vi "[ex ce] Simple Waveform Processing.vi"() -> ()   [LabVIEW 2021]
doc: "In this example, CalcExpress.vi is used for simple processing of waveform signals.\n\n::: CalcExpress Toolkit :::\nCopyright (c) 2000-2026 Konstantin Shifershteyn. All rights reserved."
uses:
  <vilib>/measure/NI_MABase.lvlib
panel:
  out "Output signals":waveform(dbl)[](graph)
  in  "Expression":string="Out1 = (In1 + In2) / 2;  // calculate average of two input signals\nOut2 = (Out1 > 1.25);    // compare the average with a threshold\n\nOut3 = (In1 > In2);      // compare two signals\nOut3 -= 2;               // substract 2 from Out3"
  out "Input signals":waveform(dbl)[](graph)
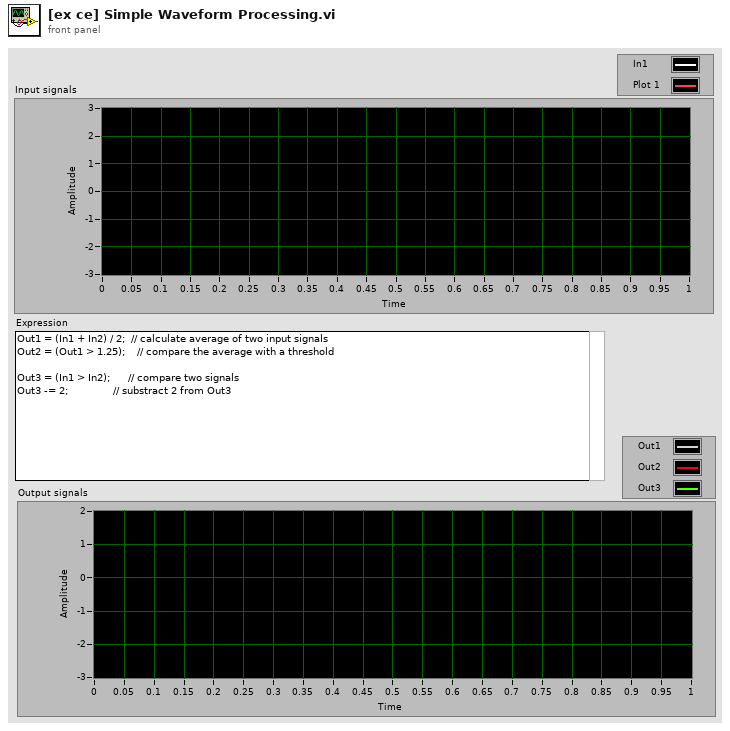
[diagram p1: front panel]
types:
  T1 = typedef "VarMan Variable Context Handle.ctl" = i32
  T2 = enum16{"create", "destroy", "set value", "get value"}
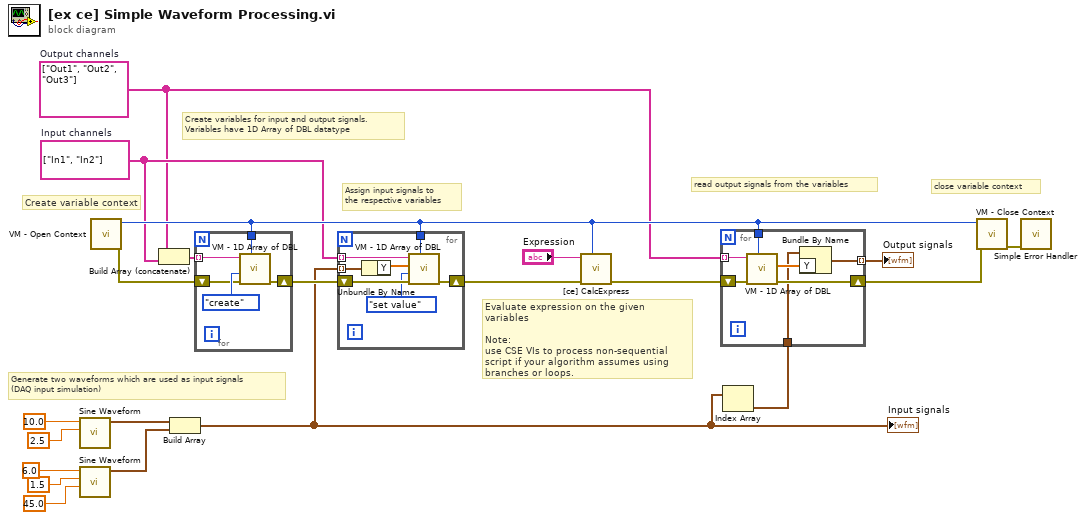
[diagram p0: block diagram]
diagram:
  w7 = string[] ["Out1", "Out2", "Out3"]  # Output channels
  w9 = string[] ["In1", "In2"]  # Input channels
  # "Create variables for input and output signals.\nVariables have 1D Array of DBL datatype"
  # "Evaluate expression on the given variables\n\nNote:\nuse CSE VIs to process non-sequential\nscript if your algorithm assumes using\nbranches or loops."
  # "close variable context"
  # "read output signals from the variables"
  # "Assign input signals to\nthe respective variables"
  # "Create variable context"
  # "Generate two waveforms which are used as input signals\n(DAQ input simulation)"
  n1 = call <vilib>:"Sine Waveform.vi"("amplitude"=2.5, "frequency"=10.0) -> ("signal out"=w16:waveform(dbl))  [unwired: 8 in, 1 out]
  n2 = call <vilib>:"Sine Waveform.vi"("phase"=45.0, "amplitude"=1.5, "frequency"=6.0) -> ("signal out"=w13:waveform(dbl))  [unwired: 7 in, 1 out]
  n3 = call "VM - Open Context.vi"() -> ("error out"=w20:errorcluster, "VC Handle out"=w11:T1)  [unwired: 9 in, 1 out]
  n4 = Build Array (concatenate)(w7, w9) -> (w8:string[])
  n5 = Build Array(w16, w13) -> (w4:waveform(dbl)[])
  "Input signals" <- w4
  n6 = for {
    shift-right: [w24] -> w14
    shift-left: w20 -> [w25]
    tunnel: w11 -> [w23]
    tunnel: w8 -> [w22] mode=indexing
    n7 = call "VM - 1D Array of DBL.vi"("VC Handle"=w23, "error in"=w25, "cmd"=T2."create", "name_spec"=w22) -> ("error out"=w24:errorcluster)  [unwired: 2 in, 5 out]
  }
  n8 = for {
    tunnel: w11 -> [w31]
    shift-right: [w30] -> w10
    shift-left: w14 -> [w33]
    tunnel: w9 -> [w29] mode=indexing
    tunnel: w4 -> [w27] mode=indexing
    n9 = Unbundle By Name(w27) -> ("Y"=w28:dbl[])
    n10 = call "VM - 1D Array of DBL.vi"("VC Handle"=w31, "error in"=w33, "cmd"=T2."set value", "value in"=w28, "name_spec"=w29) -> ("error out"=w30:errorcluster)  [unwired: 1 in, 5 out]
  }
  n11 = call "[ce] CalcExpress.vi"("VC Handle"=w11, "error in"=w10, "expression"="Expression") -> ("error out"=w12:errorcluster)  [unwired: 3 in, 3 out]
  n12 = Index Array(array=w4) -> (element=w3:waveform(dbl))  [unwired: 1 in]
  n13 = for {
    tunnel: w11 -> [w39]
    shift-right: [w37] -> w6
    shift-left: w12 -> [w40]
    tunnel: w7 -> [w36] mode=indexing
    tunnel: [w35] -> w5 mode=indexing
    tunnel: w3 -> [w34]
    n14 = call "VM - 1D Array of DBL.vi"("VC Handle"=w39, "error in"=w40, "name_spec"=w36) -> ("error out"=w37:errorcluster, "value out"=w38:dbl[])  [unwired: 3 in, 4 out]
    n15 = Bundle By Name(cluster=w34, "Y"=w38) -> (w35:waveform(dbl))
  }
  "Output signals" <- w5
  n16 = call "VM - Close Context.vi"("error in"=w6, "VC Handle"=w11) -> ("error out"=w1:errorcluster)  [unwired: 8 in, 1 out]
  n17 = call <vilib>:"Simple Error Handler.vi"("error in (no error)"=w1) -> ()  [unwired: 4 in, 5 out]
